vi "GAP_AcquireImagesV2_0.vi"() -> ()   [LabVIEW 2020]
uses:
  <vilib>/vision/driver/IMAQdx.llb/IMAQdx Buffer Number Mode.ctl
  <vilib>/vision/driver/NI_Vision_Acquisition_Software.lvlib
  <vilib>/vision/NI_Vision_Development_Module.lvlib
  <resource>/objmgr/imaqdx.rc
panel:
  out "Numeric":i32
  in  "Tab Control":T1(tab)
  in  "Camera Name":refnum<k21> caption="IMAQdx Session"
  out "Original Image":T2(plugin-control)
  out "Grayscale Image":T2(plugin-control)
  out "Acquired imgs":u32
  out "Frame rate":dbl
  in  "Overwrite Mode":u16(ring) items=["Get Oldest"=0, "Fail"=2, "Get Newest"=3]
  in  "Percent of Images Reserved by Driver":dbl=50.0
  out "ROI information":T3 {"Minimum grayscale value" format="%.2f"; "Std. dev. of pixels values [ % ]" format="%.2f"; "Mean value of pixels values" format="%.2f"; "Maximum grayscale value" format="%.2f"}
  out "Line Profile":cluster{"x0":sgl, "dx":sgl, "Pixels Line":sgl[]}(graph)
  in  "Start acquisition":bool
  in  "Stop image acquisition":bool
  in  "Save image":bool
  in  "stop 2":bool
  in  "stop":bool
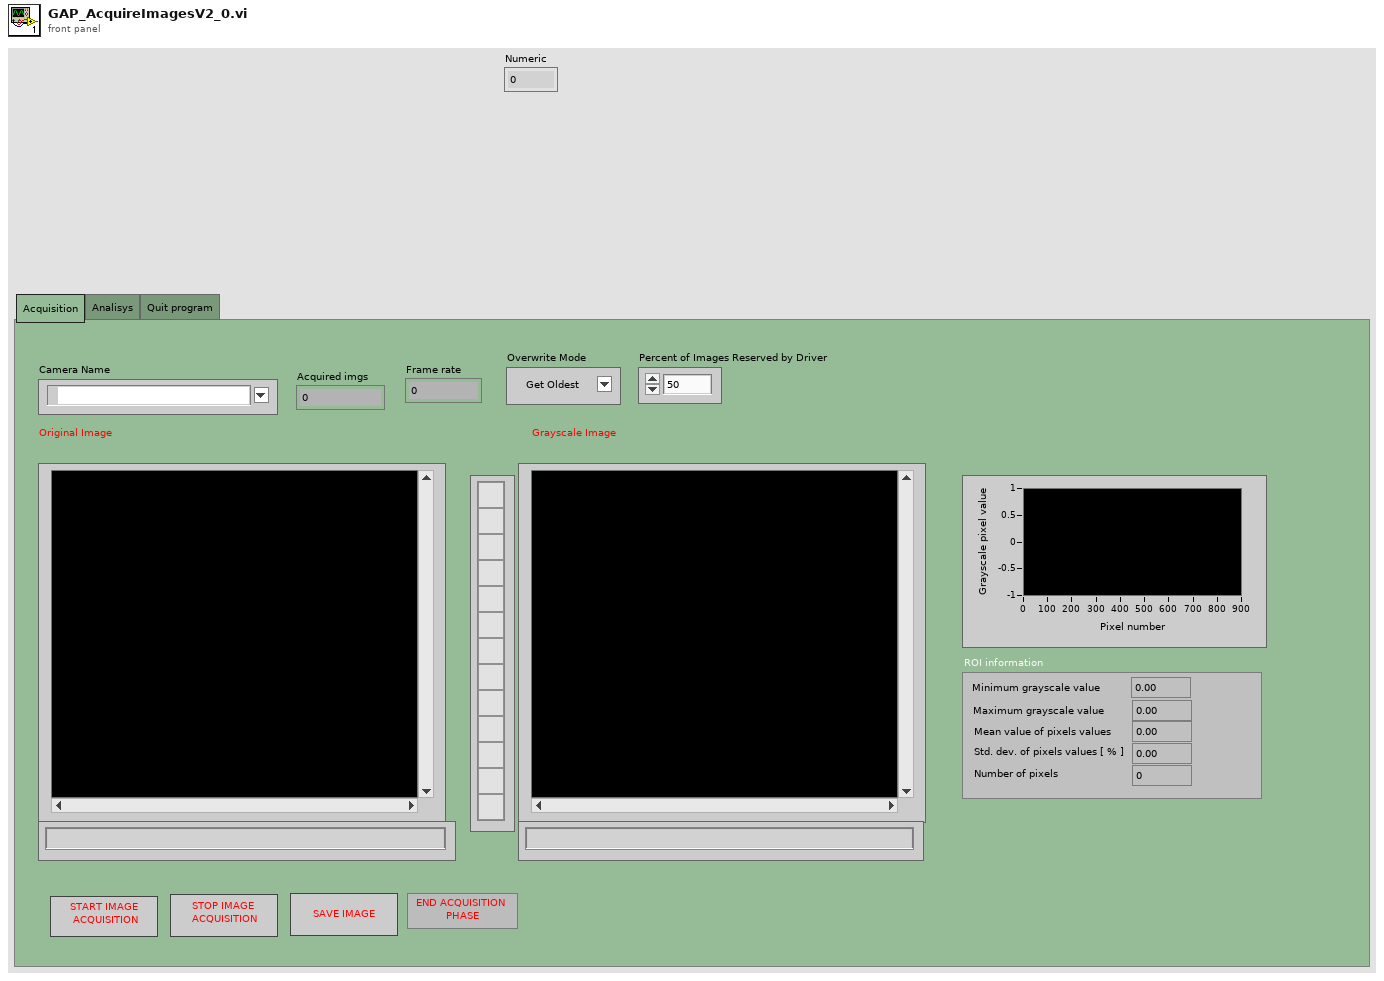
[diagram p1: front panel]
types:
  T1 = enum32{"Acquisition", "Analisys", "Quit program"}
  T2 = typedef "IMAQ Image.ctl" = refnum<image>
  T3 = cluster{"Minimum grayscale value":sgl, " Maximum grayscale value":sgl, "Mean value of pixels values":sgl, "Std. dev. of pixels values [ % ]":sgl, "Number of pixels":i32}
  T4 = typedef "NI_Vision_Acquisition_Software.lvlib/IMAQdx Buffer Number Mode.ctl" = enum32{"Next", "Last", "Buffer Number", "Every", "Last New"}
  T5 = typedef "Image Type" = u32
  T6 = typedef "IMAQdx.ctl" = refnum<k21>
  T7 = cluster{"Min":sgl, "Max":sgl, "Mean":sgl, "Std Dev":sgl, "Count":i32}
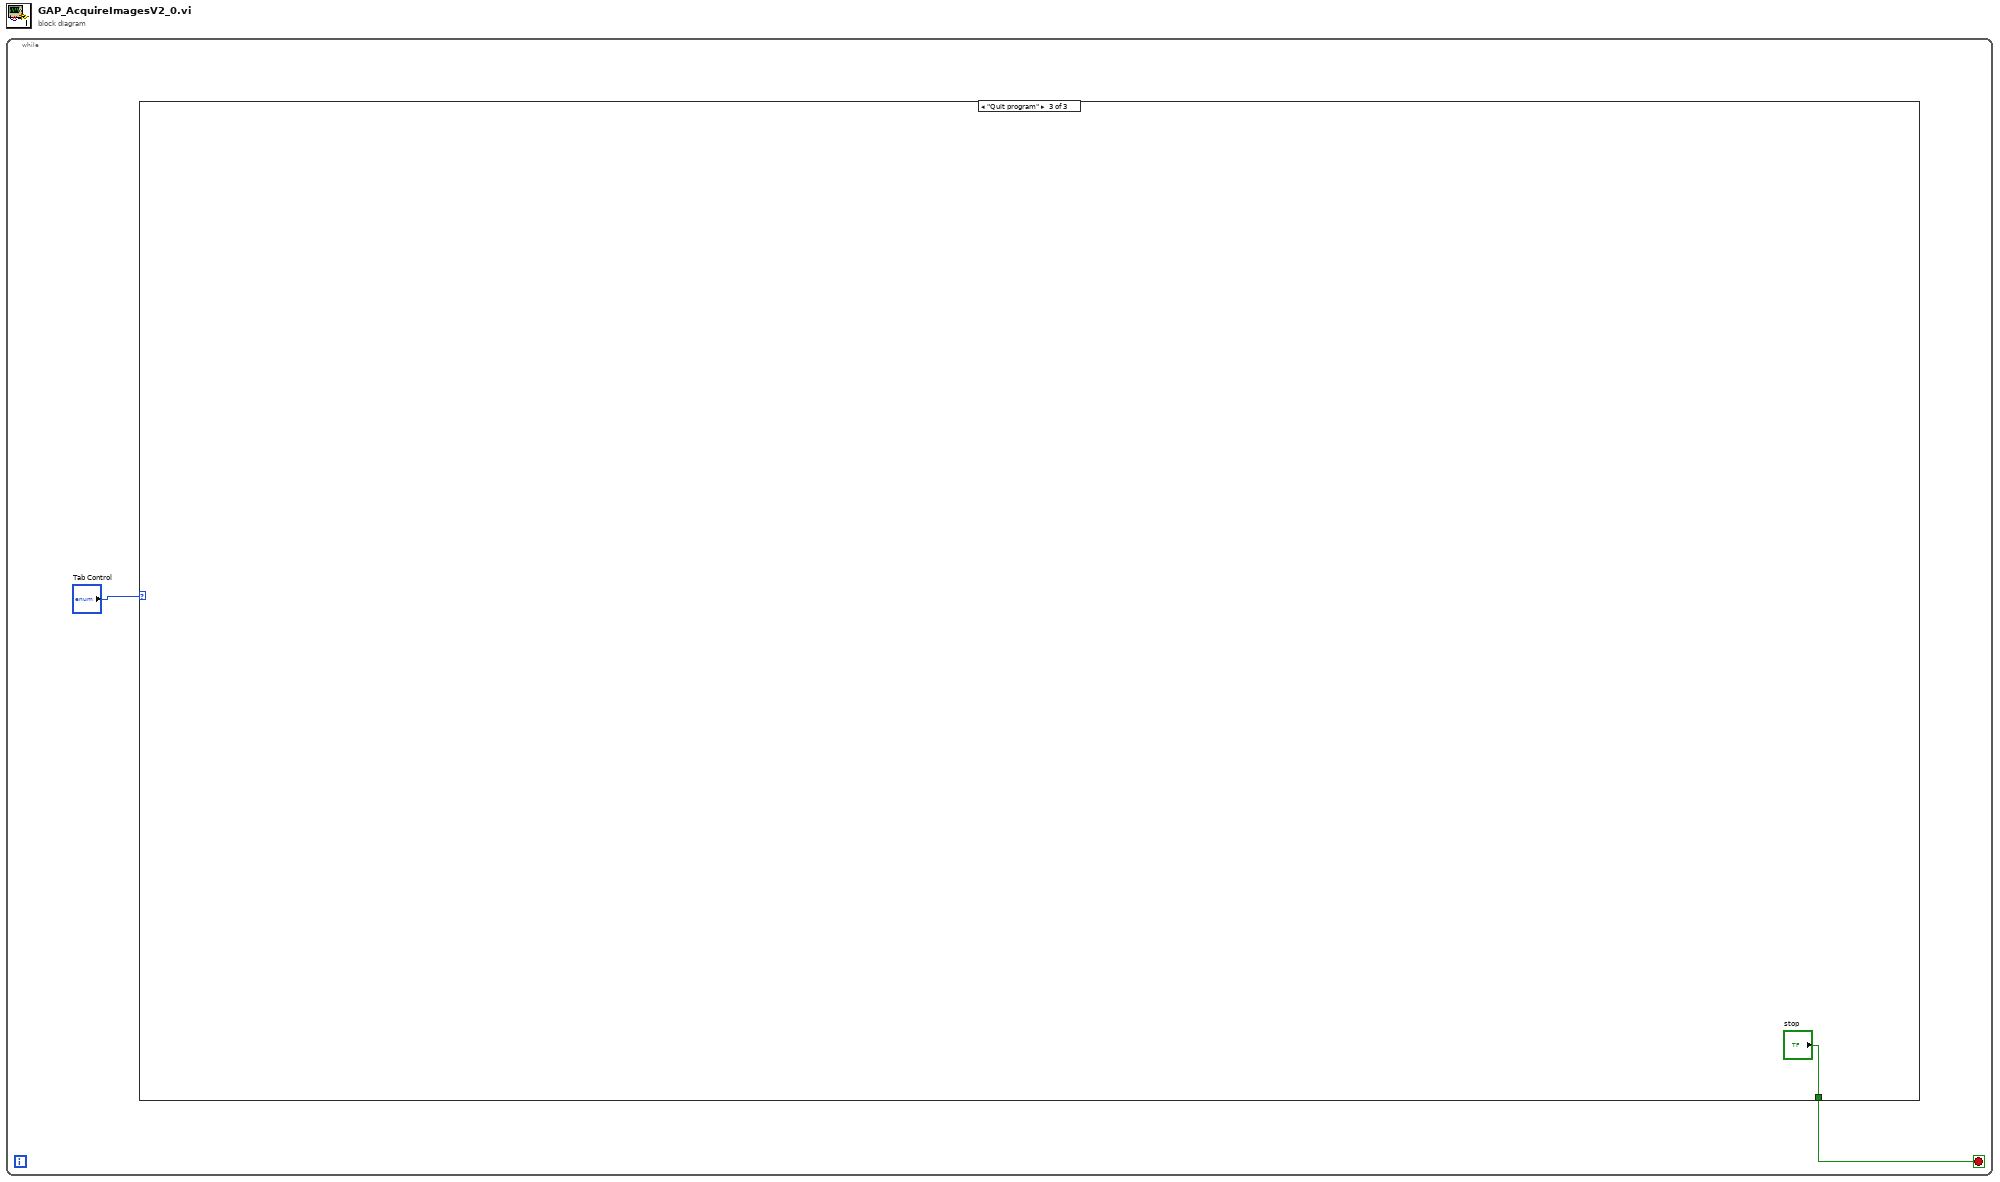
[diagram p0: block diagram]
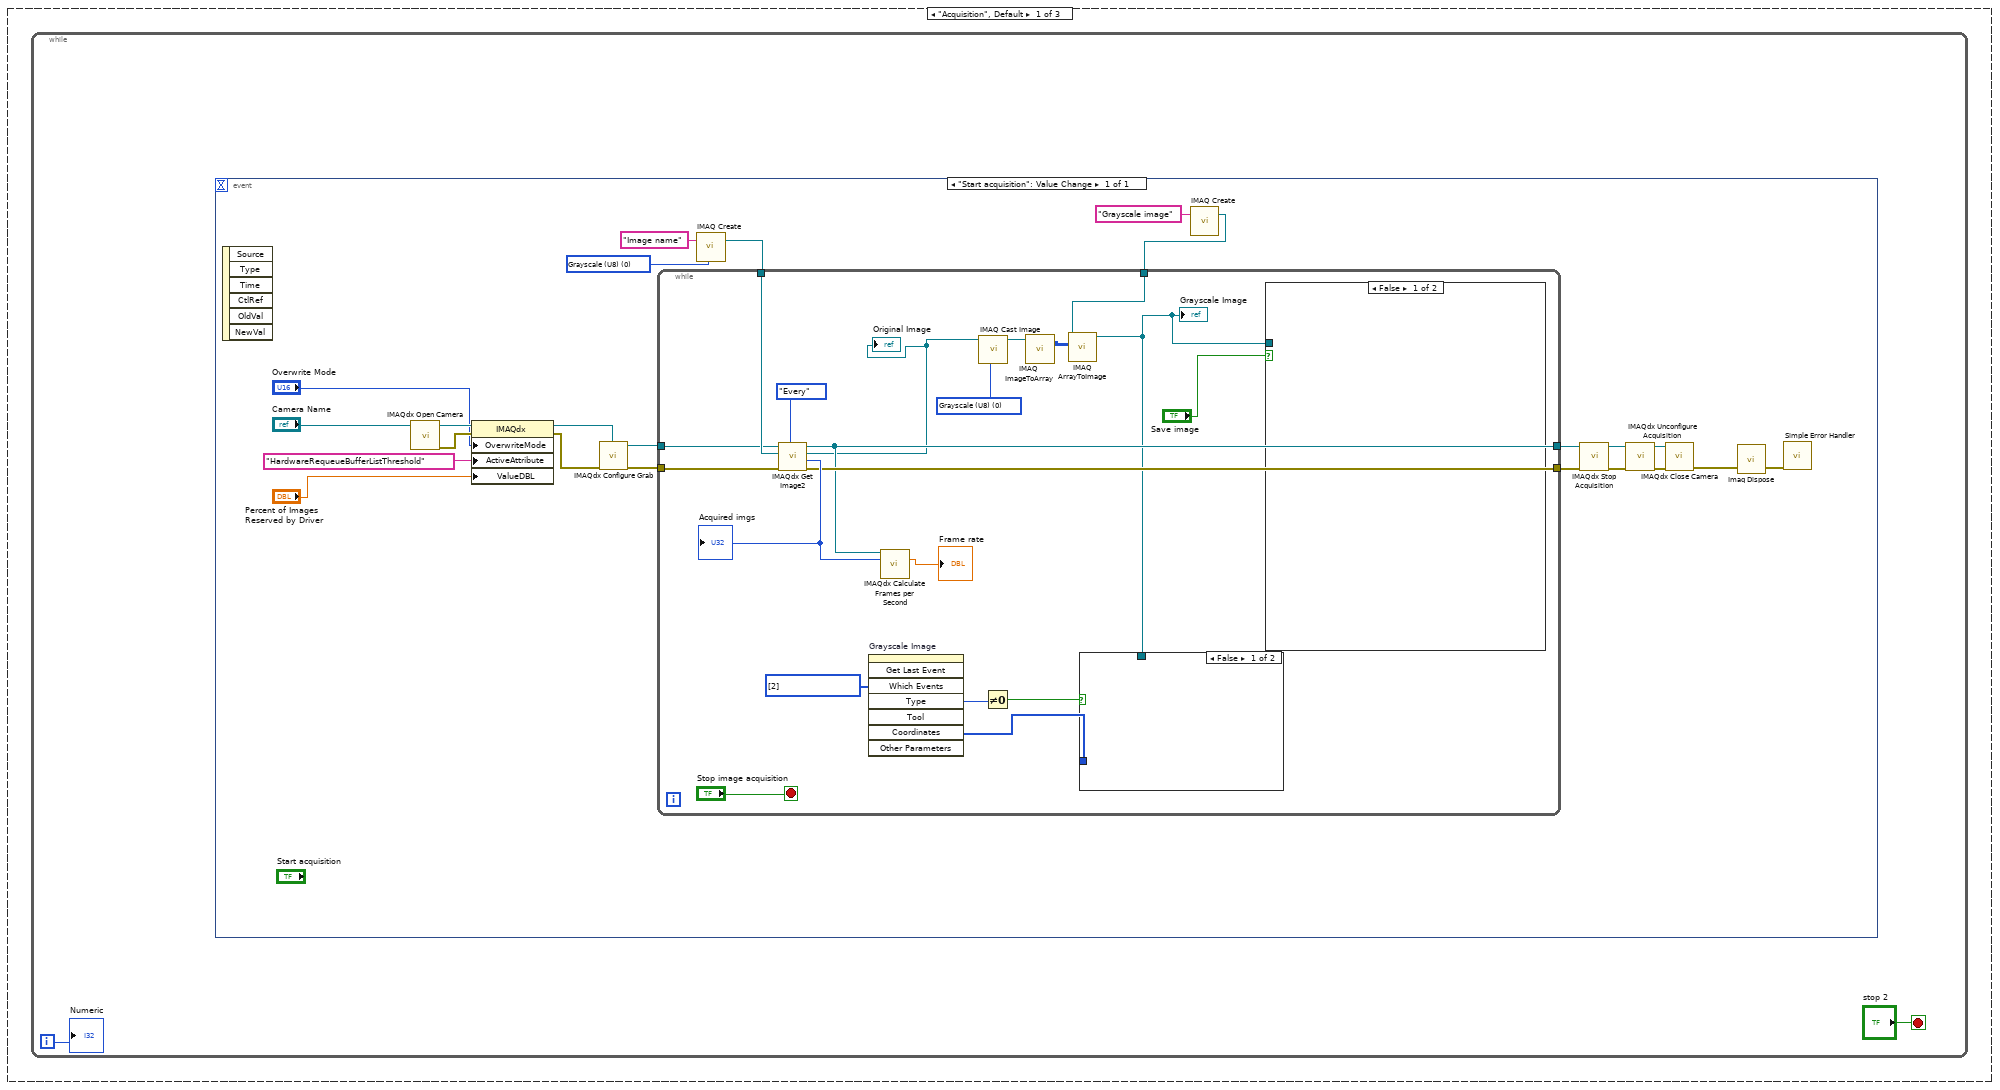
[diagram p2: hidden frame]
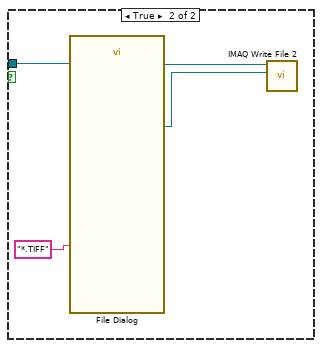
[diagram p3: hidden frame]
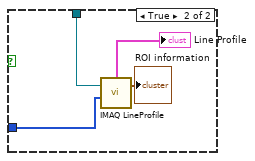
[diagram p4: hidden frame]
diagram:
  n1 = while {
    stop <- w1 stop-if-true
    n2 = case shown="\"Quit program\"" "Tab Control" {
      tunnel: [_ _ "stop"] -> w1
      frame "Acquisition", Default {
        n3 = while {
          i -> [w3]
          stop <- "stop 2" stop-if-true
          n4 = event shown="[0] \"Start acquisition\": Value Change" {
            selector: _ -> [_]
            dyn-events: _ -> [_]
            timeout: _ -> [_]
            event "Start acquisition": Value Change {
              w5 = T5 0 items=["Grayscale (U8)", "Grayscale (I16)", "Grayscale (SGL)", "Complex (CSG)", "RGB (U32)", "HSL (U32)", "RGB (U64)", "Grayscale (U16)"] ("Image Type")
              n5 = event-data() -> ()  [unwired: 1 in, 6 out]
              n6 = call <vilib>:"IMAQdx Open Camera.vi"("Session In"="Camera Name") -> ("error out"=w24:errorcluster, "Session Out"=w25:T6)  [unwired: 2 in, 7 out]
              n7 = property class="IMAQdx"(reference=w25, error in=w24, "OverwriteMode"="Overwrite Mode", "ActiveAttribute"="HardwareRequeueBufferListThreshold", "ValueDBL"="Percent of Images Reserved by Driver") -> (reference out=w20:T6, error out=w21:errorcluster)
              n8 = call <vilib>:"IMAQdx Configure Grab.vi"("error in"=w21, "Session In"=w20) -> ("error out"=w18:errorcluster, "Session Out"=w19:T6)  [unwired: 8 in]
              n9 = call "IMAQ Create"("Image Name"="Image name", "Image Type"=w5) -> ("New Image"=w16:T2)  [unwired: 2 in, 2 out]
              n10 = call "IMAQ Create"("Image Name"="Grayscale image") -> ("New Image"=w6:T2)  [unwired: 3 in, 2 out]
              n11 = while {
                tunnel: w16 -> [w46]
                tunnel: w19 -> [w44]
                tunnel: w18 -> [w43]
                tunnel: [w42] -> w9
                tunnel: [w41] -> w8
                tunnel: w6 -> [w31]
                stop <- "Stop image acquisition" stop-if-true
                w34 = T5 0 items=["Grayscale (U8)", "Grayscale (I16)", "Grayscale (SGL)", "Complex (CSG)", "RGB (U32)", "HSL (U32)", "RGB (U64)", "Grayscale (U16)"] ("Image Type")
                w40 = i32[] [2] items=["No Event"=0, "Click Event"=1, "Draw Event"=2, "Size Event"=4, "Scroll Event"=5, "Double Click Event"=8] ("Which Events")
                n12 = call <vilib>:"IMAQdx Get Image2.vi"("Buffer Number Mode (Next)"=IMAQdx_Buffer_Number_Mode."Every", "error in"=w43, "Image In"=w46, "Session In"=w44) -> ("error out"=w42:errorcluster, "Buffer Number Out"=w47:u32, "Image Out"=w30:T2, "Session Out"=w41:T6)  [unwired: 4 in]
                "Acquired imgs" <- w47
                "Original Image" <- w30
                n13 = invoke on="Grayscale Image" class="ImageControl" method="Get Last Event"("Which Events"=w40) -> ("Type"=w39:i32, "Coordinates"=w37:i32[])  [unwired: 7 in, 6 out]
                n14 = call <vilib>:"IMAQdx Calculate Frames per Second.vi"("Session In"=w41, "Buffer Number"=w47) -> ("Acquired Frames per Second"=→"Frame rate":dbl)  [unwired: 7 in, 6 out]
                n15 = call "IMAQ Cast Image"("Image Type"=w34, "Image Src"=w30) -> ("Image Dst Out"=w33:T2)  [unwired: 4 in, 5 out]
                n16 = Not Equal To 0?(x=w39) -> (x != 0?=w38:bool)
                n17 = call "IMAQ ImageToArray"("Image"=w33) -> ("Image Pixels (U8)"=w32:u8[][])  [unwired: 3 in, 4 out]
                n18 = call "IMAQ ArrayToImage"("Image Pixels (U8)"=w32, "Image"=w31) -> ("Image Out"=w29:T2)  [unwired: 8 in, 1 out]
                "Grayscale Image" <- w29
                n19 = case shown="False" w38 {
                  tunnel: w37 -> [_ w53]
                  tunnel: w29 -> [_ w52]
                  frame False {
                  }
                  frame True {
                    n20 = call "IMAQ LineProfile"("Line Coordinates"=w53, "Image"=w52) -> ("Line Graph"=→"Line Profile":cluster{"x0":sgl, "dx":sgl, "Pixels Line":sgl[]}, "Line Information"=→"ROI information":T7)  [unwired: 3 in, 2 out]
                  }
                }
                n21 = case shown="False" "Save image" {
                  tunnel: w29 -> [_ w50]
                  frame False {
                  }
                  frame True {
                    n22 = call "File Dialog"("pattern (all files)"="*.TIFF" ("pattern label")) -> ("selected path"=w49:path)  [unwired: 11 in, 3 out]
                    n23 = call-poly "IMAQ Write File 2"("File Path"=w49, "Image"=w50) -> ()  [unwired: 8 in, 2 out]
                  }
                }
              }
              n24 = call <vilib>:"IMAQdx Stop Acquisition.vi"("error in"=w9, "Session In"=w8) -> ("error out"=w11:errorcluster, "Session Out"=w12:T6)  [unwired: 8 out]
              n25 = call <vilib>:"IMAQdx Unconfigure Acquisition.vi"("error in"=w11, "Session In"=w12) -> ("error out"=w13:errorcluster, "Session Out"=w14:T6)  [unwired: 8 out]
              n26 = call <vilib>:"IMAQdx Close Camera.vi"("error in"=w13, "Session In"=w14) -> ("error out"=w10:errorcluster)  [unwired: 9 out]
              n27 = call "Imaq Dispose"("error in (no error)"=w10) -> ("error out"=w15:errorcluster)  [unwired: 5 in]
              n28 = call <vilib>:"Simple Error Handler.vi"("error in (no error)"=w15) -> ()  [unwired: 4 in, 5 out]
            }
          }
          "Numeric" <- w3
        }
      }
      frame "Analisys" {
      }
      frame "Quit program" {
      }
    }
  }
